vi "Unflatten Iceoryx Writer Configuration.vi"(8 "error in":errorcluster, 9 "Descriptor":string, 10 "Name":string, 11 "Custom Config Data in":u8[](array[numeric])) -> (0 "error out":errorcluster, 2 "FIFO Configuration":T1, 3 "CIF Pcap Publisher Configuration":T2, 5 "Updated Class Name":string)   [LabVIEW 2021, in "CIF_Iceoryx_PCAP_Universal.lvclass"]
uses:
  CIF_Iceoryx_PCAP_Universal.lvclass
  <vilib>/CIF Foundation/CIF Iceoryx/typedef/CIF Pcap Publisher Configuration.ctl
  Typedef/FIFO Configuration.ctl
  ChannelCommon/ChannelCommon.lvlib
  <vilib>/CIF Foundation/CIF Iceoryx/Iceoryx.lvlib
  Iceorxy Utilities/Iceoryx Channel Utilities.lvlib
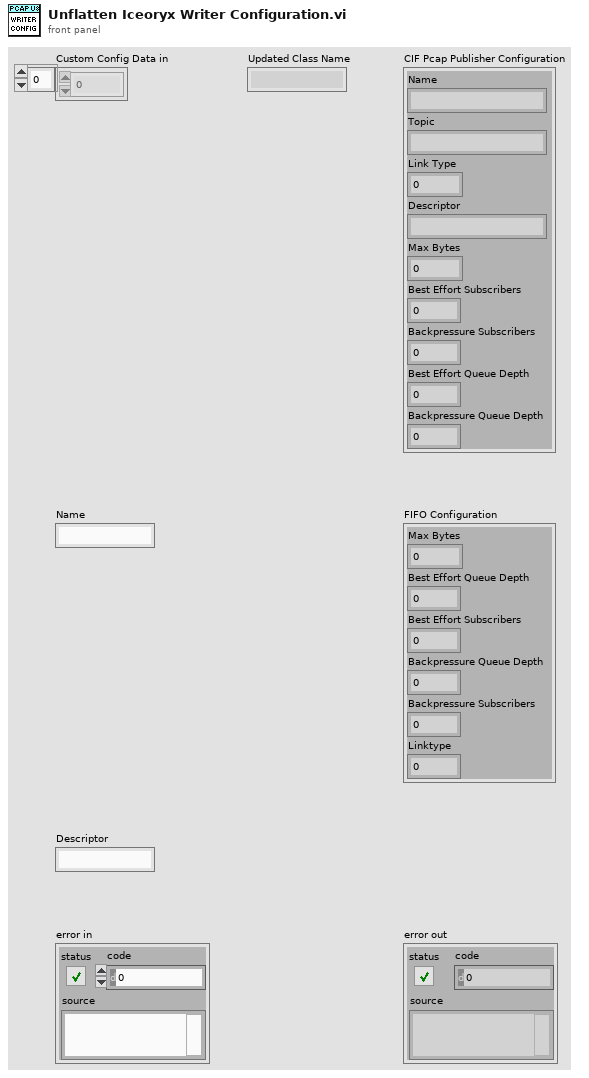
[diagram p1: front panel]
types:
  T1 = typedef "CIF_Iceoryx_PCAP_Universal.lvclass/FIFO Configuration.ctl" = cluster{"Max Bytes":u32, "Best Effort Queue Depth":u32, "Best Effort Subscribers":u32, "Backpressure Queue Depth":u32, "Backpressure Subscribers":u32, "Linktype":u32}
  T2 = typedef "Iceoryx.lvlib/CIF Pcap Publisher Configuration.ctl" = cluster{"Name":string, "Topic":string, "Link Type":u32, "Descriptor":string, "Max Bytes":u32, "Best Effort Subscribers":u32, "Backpressure Subscribers":u32, "Best Effort Queue Depth":u32, "Backpressure Queue Depth":u32}
  T3 = typedef "ChannelCommon.lvlib/FIFO Config Extended.ctl" = cluster{"Max Bytes/Msg":u64, "Max Msg/FIFO":u64, "Flags":u64, "Best Effort Subscribers":u32, "Backpressure Subscribers":u32, "Custom Data":u8[]}
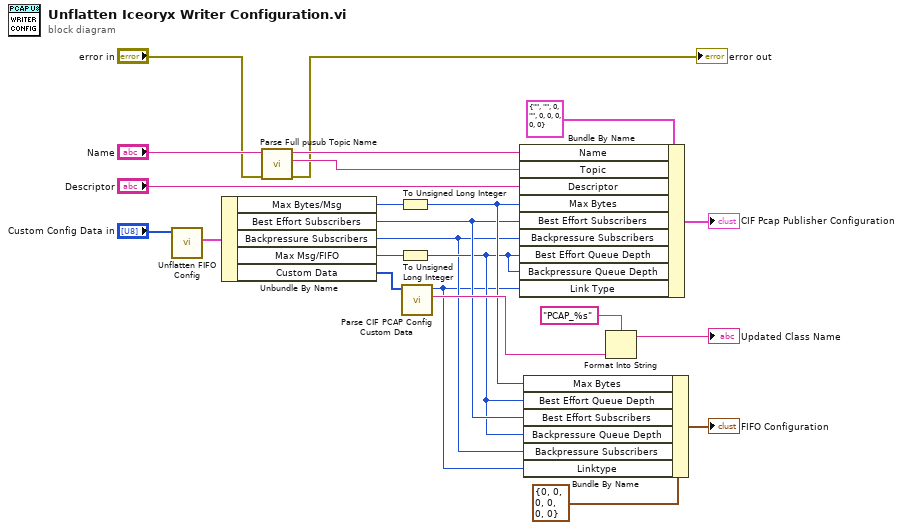
[diagram p0: block diagram]
diagram:
  n1 = call "Unflatten FIFO Config.vi"("Flattened Data in"="Custom Config Data in") -> ("FIFO Config Extended in"=w20:T3)  [unwired: 8 in, 2 out]
  n2 = Unbundle By Name(w20) -> ("Max Bytes/Msg"=w16:u64, "Best Effort Subscribers"=w5:u32, "Backpressure Subscribers"=w3:u32, "Max Msg/FIFO"=w15:u64, "Custom Data"=w8:u8[])
  n3 = call "Parse Full pusub Topic Name.vi"("error in"="error in", "Full pubsub Topic Name"="Name") -> ("error out"=→"error out":errorcluster, "Topic"=w17:string, "Plugin name"=w18:string)  [unwired: 7 in]
  n4 = To Unsigned Long Integer(number=w16) -> (unsigned 32bit integer=w6:u32)
  n5 = To Unsigned Long Integer(number=w15) -> (unsigned 32bit integer=w4:u32)
  n6 = call "Parse CIF PCAP Config Custom Data.vi"("Flattened PCAP FIFO Custom Data"=w8) -> ("Linktype Name"=w10:string, "LinkType"=w2:u32)  [unwired: 8 in, 1 out]
  n7 = Bundle By Name(cluster=T2 {"Name"="", "Topic"="", "Link Type"=0, "Descriptor"="", "Max Bytes"=0, "Best Effort Subscribers"=0, "Backpressure Subscribers"=0, "Best Effort Queue Depth"=0, "Backpressure Queue Depth"=0} ("CIF Pcap Publisher Configuration"), "Name"=w18, "Topic"=w17, "Descriptor"="Descriptor", "Max Bytes"=w6, "Best Effort Subscribers"=w5, "Backpressure Subscribers"=w3, "Best Effort Queue Depth"=w4, "Backpressure Queue Depth"=w4, "Link Type"=w2) -> (→"CIF Pcap Publisher Configuration":T2)
  n8 = Bundle By Name(cluster=T1 {"Max Bytes"=0, "Best Effort Queue Depth"=0, "Best Effort Subscribers"=0, "Backpressure Queue Depth"=0, "Backpressure Subscribers"=0, "Linktype"=0} ("FIFO Configuration"), "Max Bytes"=w6, "Best Effort Queue Depth"=w4, "Best Effort Subscribers"=w5, "Backpressure Queue Depth"=w4, "Backpressure Subscribers"=w3, "Linktype"=w2) -> (→"FIFO Configuration":T1)
  n9 = Format Into String(format string="PCAP_%s", w10) -> (resulting string=→"Updated Class Name":string)  [unwired: 2 in, 1 out]
